vi "4Pi 4Pi Modes - Write DM.vi"(0 "DM Handles":T1(array[cluster]), 1 "Error In":errorcluster, 2 "No hardware":bool=TRUE, 3 "Norm Voltage (-1, 1)":dbl[](array[numeric])) -> (6 "Error Out":errorcluster)   [LabVIEW 2016]
uses:
  <userlib>/BMC/BMC.lvlib
panel:
  out "Debug BMC Send Data":dbl[][](array[numeric])
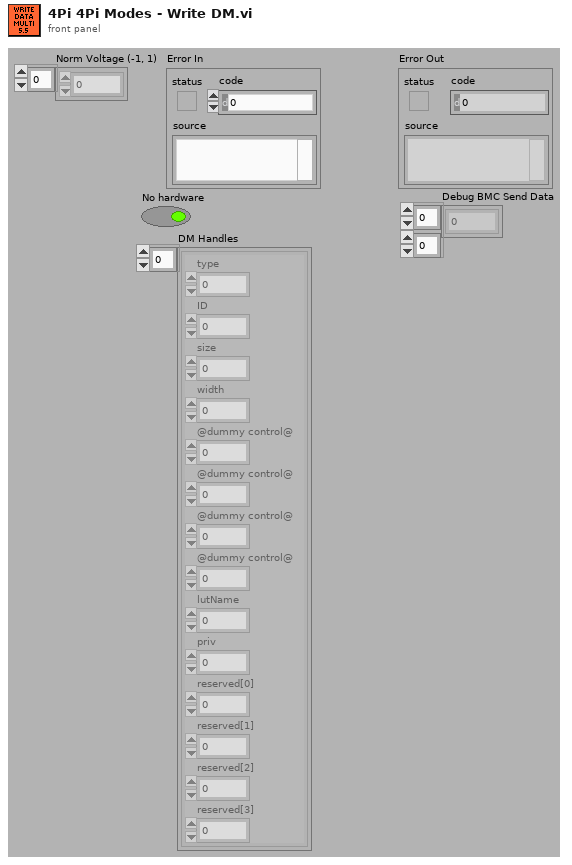
[diagram p1: front panel]
types:
  T1 = cluster{"type":i16, "ID":i16, "size":i32, "width":i32, "@dummy control@":i8, "@dummy control@":i8, "@dummy control@":i8, "@dummy control@":i8, "lutName":u64, "priv":u64, "reserved[0]":i32, "reserved[1]":i32, "reserved[2]":i32, "reserved[3]":i32}[]
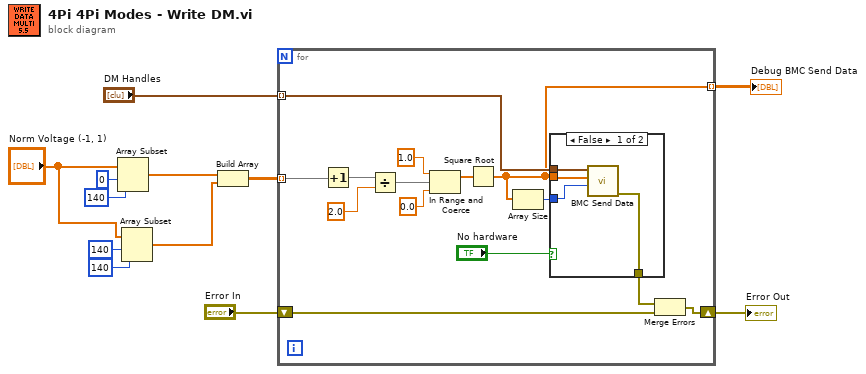
[diagram p0: block diagram]
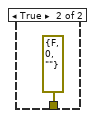
[diagram p2: hidden frame]
diagram:
  n1 = Array Subset(array="Norm Voltage (-1, 1)", index=0, length=140) -> (w7:dbl[])
  n2 = Array Subset(array="Norm Voltage (-1, 1)", index=140, length=140) -> (w6:dbl[])
  n3 = Build Array(w7, w6) -> (w5:dbl[][])
  n4 = for {
    tunnel: w5 -> [w26] mode=indexing
    tunnel: "DM Handles" -> [w20] mode=indexing
    shift-right: [w16] -> w3
    shift-left: "Error In" -> [w17]
    tunnel: [w13] -> w1 mode=indexing
    n5 = Increment(x=w26) -> (x+1=w25:dbl[])
    n6 = Divide(x=w25, y=2.0 ("x")) -> (x/y=w23:dbl[])
    n7 = In Range and Coerce(upper limit=1.0 ("x"), x=w23, lower limit=0.0 ("x")) -> (coerced(x)=w15:dbl[])  [unwired: 1 out]
    n8 = Square Root(x=w15) -> (sqrt(x)=w13:dbl[])
    n9 = Array Size(array=w13) -> (size(s)=w19:i32)
    n10 = case shown="False" "No hardware" {
      tunnel: w20 -> [w30 _]
      tunnel: w19 -> [w29 _]
      tunnel: [w28 errorcluster {"status"=FALSE, "code"=0, "source"=""} ("error out")] -> w18
      tunnel: w13 -> [w27 _]
      frame False {
        n11 = call <userlib>:"BMC Send Data.vi"("length"=w29, "data"=w27, "dmHandle"=w30) -> ("error out"=w28:errorcluster)  [unwired: 7 in, 1 out]
      }
      frame True {
      }
    }
    n12 = Merge Errors(w18, w17) -> (w16:errorcluster)
  }
  "Error Out" <- w3
  "Debug BMC Send Data" <- w1
